vi "Configure_DAC_Measurement_Device.vi"(0 "Measurement Device":refnum<k15>, 5 "Current Limit":dbl, 7 "Voltage Level Range":dbl, 9 "Output Function":T1 items=["DC Voltage"=1006, "DC Current"=1007, "Pulse Voltage"=1049, "Pulse Current"=1050, "Constant Resistance"=1161, "Constant Power"=1162], 11 "Error In":errorcluster) -> (4 "Instrument Handle":refnum<k15> caption="Instrument Handle Out", 15 "Error Out":errorcluster)   [LabVIEW 2026, in "Core.lvlib"]
doc: "Initializes and configures the measurement device used to acquire DAC output values during DAC INL/DNL testing."
uses:
  Core.lvlib
  <instrlib>/niDCPower/nidcpower.llb/niDCPower Output Function.ctl
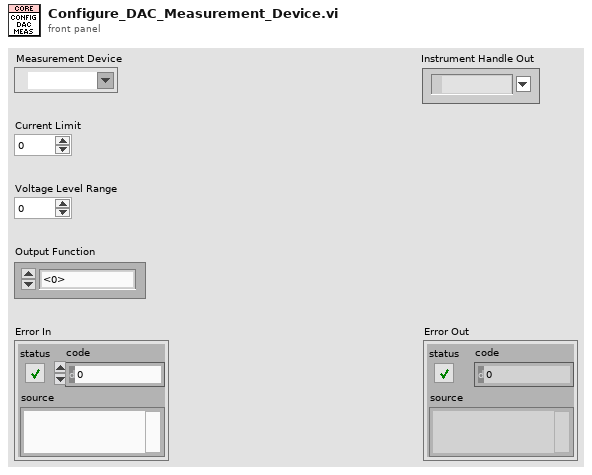
[diagram p1: front panel]
types:
  T1 = typedef "niDCPower Output Function.ctl" = i32
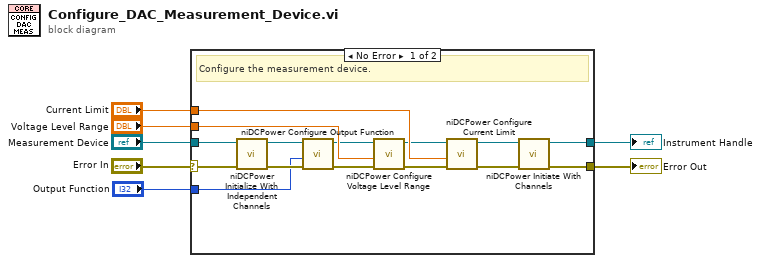
[diagram p0: block diagram]
diagram:
  n1 = case shown="No Error" "Error In" {
    selector: "Error In" -> [w22 w23]
    tunnel: "Current Limit" -> [w19 _]
    tunnel: "Voltage Level Range" -> [w18 _]
    tunnel: "Measurement Device" -> [w17 w24]
    tunnel: "Output Function" -> [w10 _]
    tunnel: [w9 w23] -> w2
    tunnel: [w8 w24] -> w1
    frame No Error {
      # "Configure the measurement device."
      n2 = call <instrlib>:"niDCPower Initialize With Independent Channels.vi"("error in (no error)"=w22, "resource name"=w17) -> ("error out"=w12:errorcluster, "instrument handle out"=w11:refnum<k15>)  [unwired: 8 in]
      n3 = call <instrlib>:"niDCPower Configure Output Function.vi"("error in (no error)"=w12, "output function"=w10, "instrument handle"=w11) -> ("error out"=w13:errorcluster, "instrument handle out"=w15:refnum<k15>)  [unwired: 7 in]
      n4 = call <instrlib>:"niDCPower Configure Voltage Level Range.vi"("error in (no error)"=w13, "voltage level range"=w18, "instrument handle"=w15) -> ("error out"=w14:errorcluster, "instrument handle out"=w16:refnum<k15>)  [unwired: 7 in]
      n5 = call <instrlib>:"niDCPower Configure Current Limit.vi"("error in (no error)"=w14, "current limit"=w19, "instrument handle"=w16) -> ("error out"=w20:errorcluster, "instrument handle out"=w21:refnum<k15>)  [unwired: 7 in]
      n6 = call <instrlib>:"niDCPower Initiate With Channels.vi"("error in (no error)"=w20, "instrument handle"=w21) -> ("error out"=w9:errorcluster, "instrument handle out"=w8:refnum<k15>)  [unwired: 8 in]
    }
    frame Error {
    }
  }
  "Error Out" <- w2
  "Instrument Handle" <- w1
